vi "Utility - Set Category List Text & Icons.vi"(8 "error in":errorcluster, 11 "LstBox Refnum":refnum<vi>) -> (0 "error out":errorcluster)   [LabVIEW 2014]
doc: "::: VI Helpeks :::\nCopyright (c) 2000-2026 Konstantin Shifershteyn. All rights reserved."
panel:
  # "VI Helpeks\nCopyright (c) 2012-2026 Konstantin Shifershteyn"
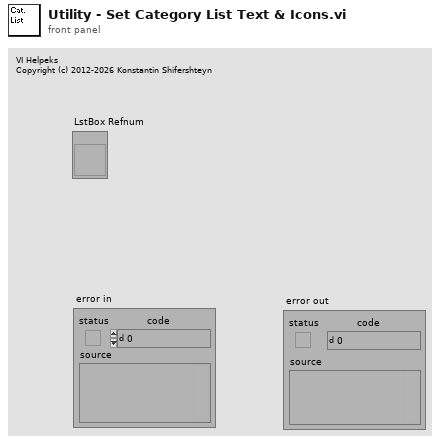
[diagram p1: front panel]
types:
  T1 = typedef "imagedata.ctl" = cluster{"image type":i32, "image depth":i32, "image":u8[], "mask":u8[], "colors":u32[], "Rectangle":cluster{"left":i16, "top":i16, "right":i16, "bottom":i16}}
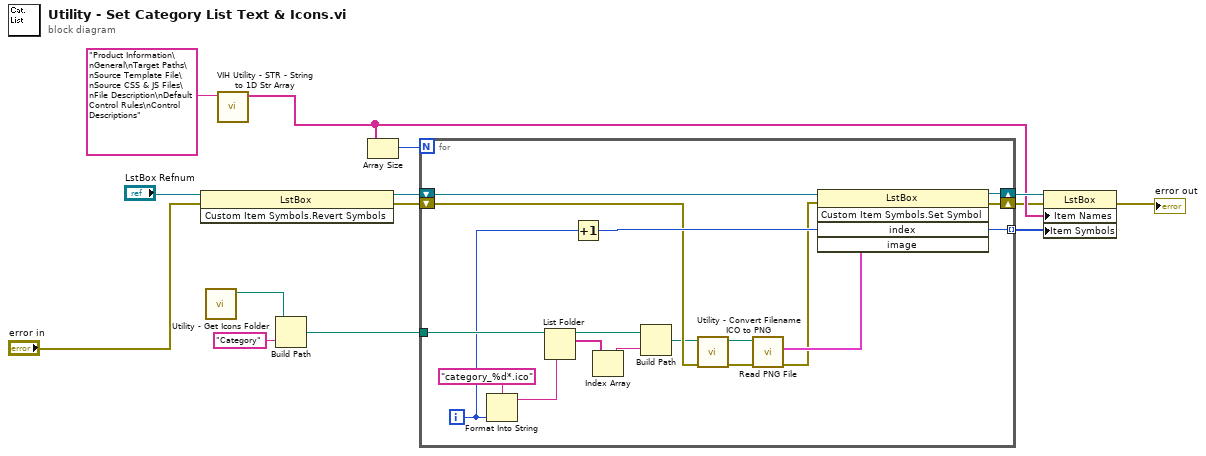
[diagram p0: block diagram]
diagram:
  n1 = invoke class="LstBox" method="Custom Item Symbols.Revert Symbols"(reference="LstBox Refnum", error in="error in") -> (reference out=w5:refnum<vi>, error out=w3:errorcluster)  [unwired: 1 in, 1 out]
  n2 = call "Utility - Get Icons Folder.vi"() -> ("Icons Folder"=w13:path)  [unwired: 10 in, 1 out]
  n3 = call "VIH Utility - STR - String to 1D Str Array.vi"("String in"="Product Information\nGeneral\nTarget Paths\nSource Template File\nSource CSS & JS Files\nFile Description\nDefault Control Rules\nControl Descriptions" ("String out")) -> ("Array out"=w6:string[])  [unwired: 6 in]
  n4 = Build Path(base path=w13, name or relative path="Category") -> (appended path=w10:path)
  n5 = Array Size(array=w6) -> (size(s)=w11:i32)
  n6 = for {
    N: w11 -> [_]
    tunnel: w10 -> [w30]
    shift-right: [w21] -> w9
    shift-left: w5 -> [w24]
    tunnel: [w20] -> w8 mode=indexing
    shift-right: [w17] -> w2
    shift-left: w3 -> [w19]
    i -> [w23]
    n7 = Format Into String(format string="category_%d*.ico", w23) -> (resulting string=w28:string)  [unwired: 2 in, 1 out]
    n8 = List Folder(path=w30, pattern=w28) -> (path out=w27:path, filenames=w26:string[])  [unwired: 2 in, 2 out]
    n9 = Increment(x=w23) -> (x+1=w20:i32)
    n10 = Index Array(array=w26) -> (element=w25:string)  [unwired: 1 in]
    n11 = Build Path(base path=w27, name or relative path=w25) -> (appended path=w16:path)
    n12 = call "Utility - Convert Filename ICO to PNG.vi"("Path"=w16) -> ("Path 2"=w15:path)  [unwired: 10 in]
    n13 = call <vilib>:"Read PNG File.vi"("error in (no error)"=w19, "path to PNG file"=w15) -> ("error out"=w18:errorcluster, "image data"=w22:T1)  [unwired: 7 in, 1 out]
    n14 = invoke class="LstBox" method="Custom Item Symbols.Set Symbol"(reference=w24, error in=w18, "index"=w20, "image"=w22) -> (reference out=w21:refnum<vi>, error out=w17:errorcluster)  [unwired: 1 in, 3 out]
  }
  n15 = property class="LstBox"(reference=w9, error in=w2, "Item Names"=w6, "Item Symbols"=w8) -> (error out=→"error out":errorcluster)  [unwired: 1 out]
